vi "Fix Read Op Value.vi"(8 "error in (no error)":errorcluster, 10 "VI Refs":refnum<vi>[](array[refnum]), 11 "Subsystem Name":string) -> (0 "error in (no error) 2":errorcluster)   [LabVIEW 2023]
uses:
  <vilib>/Utility/traverseref.llb/TRef TravTarget.ctl
  <vilib>/Utility/traverseref.llb/VI Scripting - Traverse.lvlib
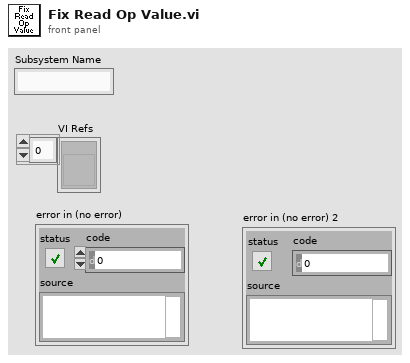
[diagram p1: front panel]
types:
  T1 = typedef "TRef TravTarget.ctl" = enum16{"FP", "BD", "Other"}
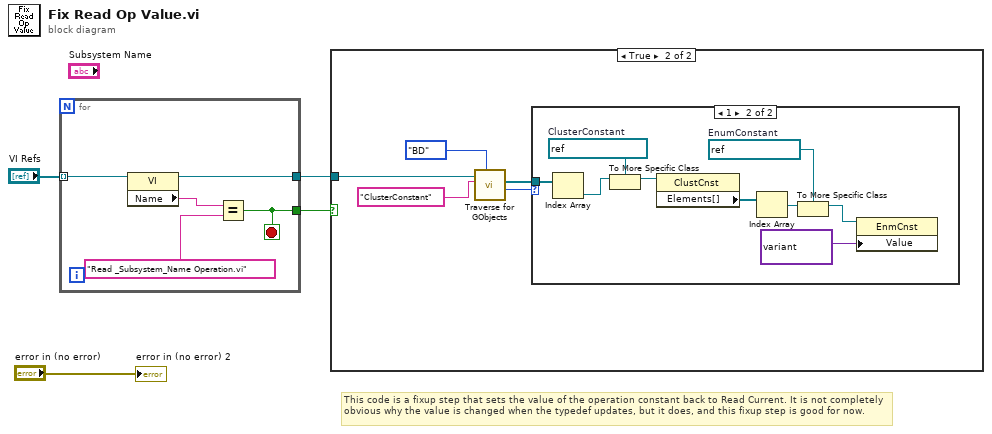
[diagram p0: block diagram]
diagram:
  # "This code is a fixup step that sets the value of the operation constant back to Read Current. It is not completely\nobvious why the value is changed when the typedef updates, but it does, and this fixup step is good for now."
  n1 = for {
    tunnel: "VI Refs" -> [w9] mode=indexing
    tunnel: [w6] -> w1
    tunnel: [w8] -> w2
    stop <- w6 stop-if-true
    n2 = property class="VI"(reference=w9) -> (reference out=w8:refnum<vi>, "Name"=w7:string)  [unwired: 1 in, 1 out]
    n3 = Equal?(x=w7, y="Read _Subsystem_Name Operation.vi") -> (x = y?=w6:bool)
  }
  n4 = case shown="True" w1 {
    tunnel: w2 -> [_ w10]
    frame False {
    }
    frame True {
      n5 = call <vilib>:"Traverse for GObjects.vi"("Traverse Target"=TRef_TravTarget."BD", "Class Name"="ClusterConstant", "VI Refnum"=w10) -> ("# of Refs"=w12:i32, "References"=w11:refnum<vi>[])  [unwired: 5 in, 2 out]
      n6 = case shown="1" w12 {
        tunnel: w11 -> [_ w23]
        frame 0, Default {
        }
        frame 1 {
          w18 = refnum<vi> refnum  # EnumConstant
          w22 = refnum<vi> refnum  # ClusterConstant
          n7 = Index Array(array=w23) -> (element=w17:refnum<vi>)  [unwired: 1 in]
          n8 = To More Specific Class(target class=w22, reference=w17) -> (specific class reference=w16:refnum<vi>)  [unwired: 1 in, 1 out]
          n9 = property class="ClustCnst"(reference=w16) -> ("Elements[]"=w21:refnum<vi>[])  [unwired: 1 in, 2 out]
          n10 = Index Array(array=w21) -> (element=w20:refnum<vi>)  [unwired: 1 in]
          n11 = To More Specific Class(target class=w18, reference=w20) -> (specific class reference=w19:refnum<vi>)  [unwired: 1 in, 1 out]
          n12 = property class="EnmCnst"(reference=w19, "Value"=variant(enum16{"Reserve", "Read Current", "Immediate"} enum."Read Current")) -> ()  [unwired: 1 in, 2 out]
        }
      }
    }
  }
  "error in (no error) 2" <- "error in (no error)"
